vi "DSS-Tests-flatten_complex.vi"(11 "values":cdb[](array[numeric])) -> (3 "flat":dbl[](array[numeric]))   [LabVIEW 2020, in "DSS-Tests.lvlib"]
doc: "Flattens a 1D complex DBL array into one 1D DBL array: the length, then all real parts, then all imaginary parts."
uses:
  DSS-Tests.lvlib
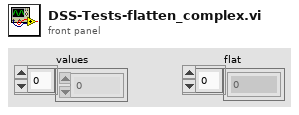
[diagram p1: front panel]
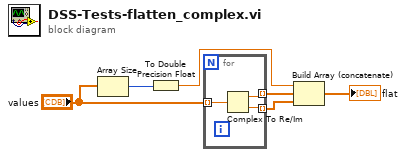
[diagram p0: block diagram]
diagram:
  n1 = Array Size(array="values") -> (size(s)=w2:i32)
  n2 = To Double Precision Float(number=w2) -> (double precision float=w3:dbl)
  n3 = for {
    tunnel: "values" -> [w7] mode=indexing
    tunnel: [w8] -> w4 mode=indexing
    tunnel: [w9] -> w5 mode=indexing
    n4 = Complex To Re/Im ("Complex To Cartesian.vi")(x + iy=w7) -> (x=w8:dbl, y=w9:dbl)
  }
  n5 = Build Array (concatenate)(w3, w4, w5) -> (→"flat":dbl[])
